vi "Read Read Only.vi"(8 "error in (no error)":errorcluster, 11 "CTI_GPIO_DigitalOut in":refnum<class "CTI_AnalogIn.lvclass">) -> (0 "error out":errorcluster, 2 "Read Only":bool, 3 "CTI_GPIO_DigitalOut out":refnum<class "CTI_AnalogIn.lvclass">)   [LabVIEW 2021, in "CTI_AnalogIn.lvclass"]
doc: "Abstract Data Classes 2.1.1.13\nTim Streeter - TSA\nCopyright (c) 2025, TSA"
uses:
  CTI_AnalogIn.lvclass
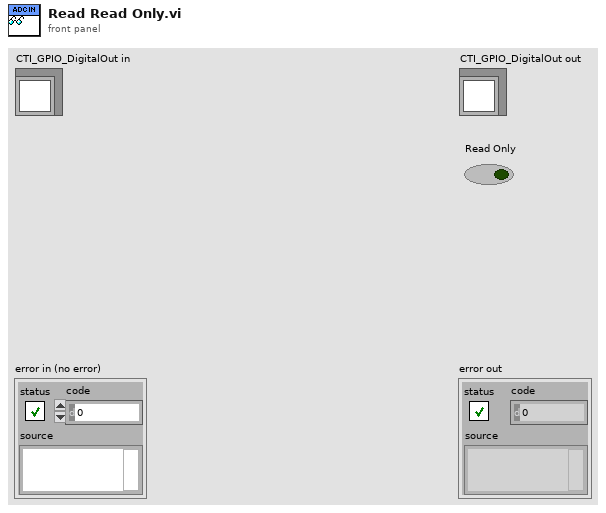
[diagram p1: front panel]
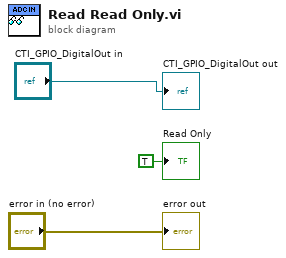
[diagram p0: block diagram]
diagram:
  "error out" <- "error in (no error)"
  "CTI_GPIO_DigitalOut out" <- "CTI_GPIO_DigitalOut in"
  "Read Only" <- TRUE ("Read Only")
